vi "Obtain Request Events.vi"(8 "error in":errorcluster, 10 "Create New? (F)":bool) -> (0 "error out":errorcluster, 2 "Sequencer Request Events":T1)   [LabVIEW 2025, in "Sequencer.lvlib"]
doc: "This VI Obtains/Creates the Requests events that will be used for other modules to communicate with the module that owns this VI. These Requests events will be accessed only via Public API methods for this module.\n\n<b>NOTE</b>: The contents of this VI are automatically generated and modified by the <b>Tools > DQMH Consortium > DQMH</b> utilities. Consider using those utilities instead of making your own modifications to this VI.\n_____\nBased on DQMH Dev Tools: Project Template 7.1.2.1547."
uses:
  Sequencer.lvlib
  Request Events--cluster.ctl
  Stop Argument--cluster.ctl
  Show Panel Argument--cluster.ctl
  Hide Panel Argument--cluster.ctl
  Show Diagram Argument--cluster.ctl
  Get Module Execution Status Argument--cluster.ctl
  Get Modules Argument--cluster.ctl
  Get Modules (Reply Payload)--cluster.ctl
  Home Argument--cluster.ctl
  Home (Reply Payload)--cluster.ctl
  Home Stepper Argument--cluster.ctl
  Home Stepper (Reply Payload)--cluster.ctl
  Go To Angle Argument--cluster.ctl
  Controls/Angle Indicator.ctl
  Controls/Motor Speed Slider.ctl
  Go To Angle (Reply Payload)--cluster.ctl
  Part Removal Position Argument--cluster.ctl
  Part Removal Position (Reply Payload)--cluster.ctl
  Torque Test Argument--cluster.ctl
  Controls/Sequencer/sequence array.ctl
  Controls/Sequencer/step cluster.ctl
  Torque Test (Reply Payload)--cluster.ctl
  Controls/Sequencer/results array.ctl
  Controls/Sequencer/results cluster.ctl
panel:
  # "NOTE: The contents of this VI are automatically generated and modified by the Tools > DQMH Consortium > DQMH utilities. Consider using those utilities instead of making your own modifications to this VI."
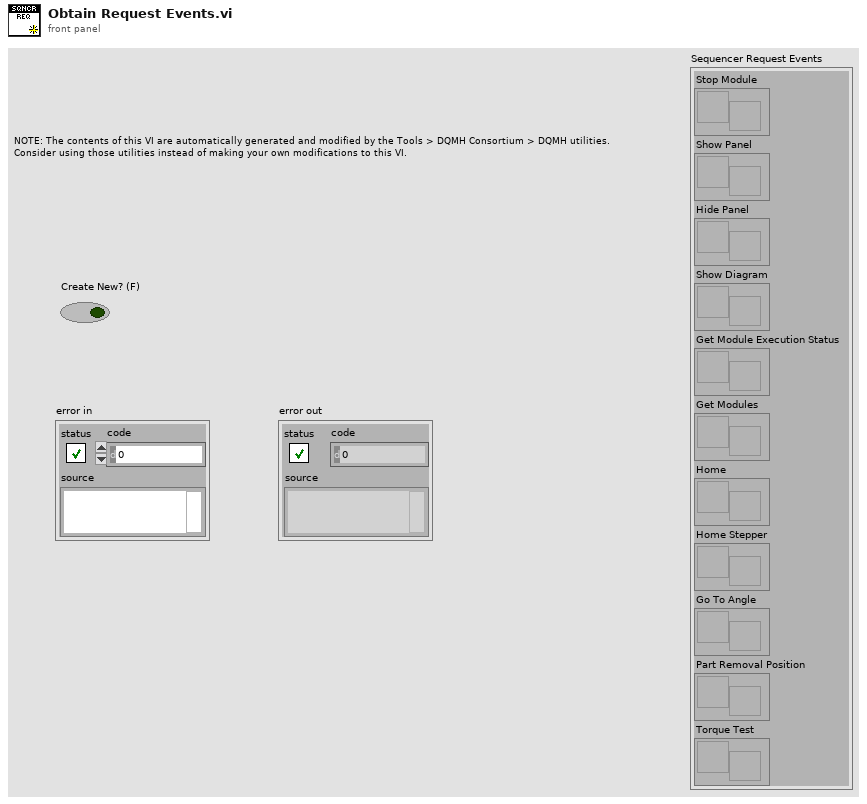
[diagram p1: front panel]
types:
  T1 = typedef "Sequencer.lvlib/Request Events--cluster.ctl" = cluster{"Stop Module":refnum<user-event>, "Show Panel":refnum<user-event>, "Hide Panel":refnum<user-event>, "Show Diagram":refnum<user-event>, "Get Module Execution Status":refnum<user-event>, "Get Modules":refnum<user-event>, "Home":refnum<user-event>, "Home Stepper":refnum<user-event>, "Go To Angle":refnum<user-event>, "Part Removal Position":refnum<user-event>, "Torque Test":refnum<user-event>}
  T2 = typedef "Sequencer.lvlib/Torque Test Argument--cluster.ctl" = cluster{"Module ID":i32, "Array 2":T3, "Speed [rpm]":T5, "On Time [ms]":dbl, "Wait Notifier":refnum<notifier>, "wait for reply":bool}
  T3 = typedef "sequence array.ctl" = T4[]
  T4 = typedef "step cluster.ctl" = cluster{"Angle Min [°]":dbl, "Angle Max [°]":dbl, "Torque Min [oz-in]":dbl, "Torque Max [oz-in]":dbl}
  T5 = typedef "Motor Speed Slider.ctl" = dbl
  T6 = typedef "Sequencer.lvlib/Part Removal Position Argument--cluster.ctl" = cluster{"Module ID":i32, "Wait Notifier":refnum<notifier>, "wait for reply":bool}
  T7 = typedef "Sequencer.lvlib/Go To Angle Argument--cluster.ctl" = cluster{"Module ID":i32, "Angle":T8, "Speed [rpm]":T5, "Wait Notifier":refnum<notifier>, "wait for reply":bool}
  T8 = typedef "Angle Indicator.ctl" = dbl
  T9 = typedef "Sequencer.lvlib/Home Stepper Argument--cluster.ctl" = cluster{"Module ID":i32, "Wait Notifier":refnum<notifier>, "wait for reply":bool}
  T10 = typedef "Sequencer.lvlib/Home Argument--cluster.ctl" = cluster{"Module ID":i32, "Wait Notifier":refnum<notifier>, "wait for reply":bool}
  T11 = typedef "Sequencer.lvlib/Get Modules Argument--cluster.ctl" = cluster{"Module ID":i32, "Modules":cluster{"Module IDs":i32[], "Module Names":string[]}, "Wait Notifier":refnum<notifier>, "wait for reply":bool}
  T12 = typedef "Sequencer.lvlib/Get Module Execution Status Argument--cluster.ctl" = cluster{"Module ID":i32, "Running?":bool}
  T13 = typedef "Sequencer.lvlib/Show Diagram Argument--cluster.ctl" = cluster{"Module ID":i32, "Debug?":bool}
  T14 = typedef "Sequencer.lvlib/Show Panel Argument--cluster.ctl" = cluster{"Module ID":i32, "Show Panel?":bool}
  T15 = typedef "Sequencer.lvlib/Hide Panel Argument--cluster.ctl" = cluster{"Module ID":i32, "Hide Panel?":bool}
  T16 = typedef "Sequencer.lvlib/Stop Argument--cluster.ctl" = cluster{"Module ID":i32, "Origin":string, "Exit via Stop Module Req?":bool, "Wait for Module to stop?":bool}
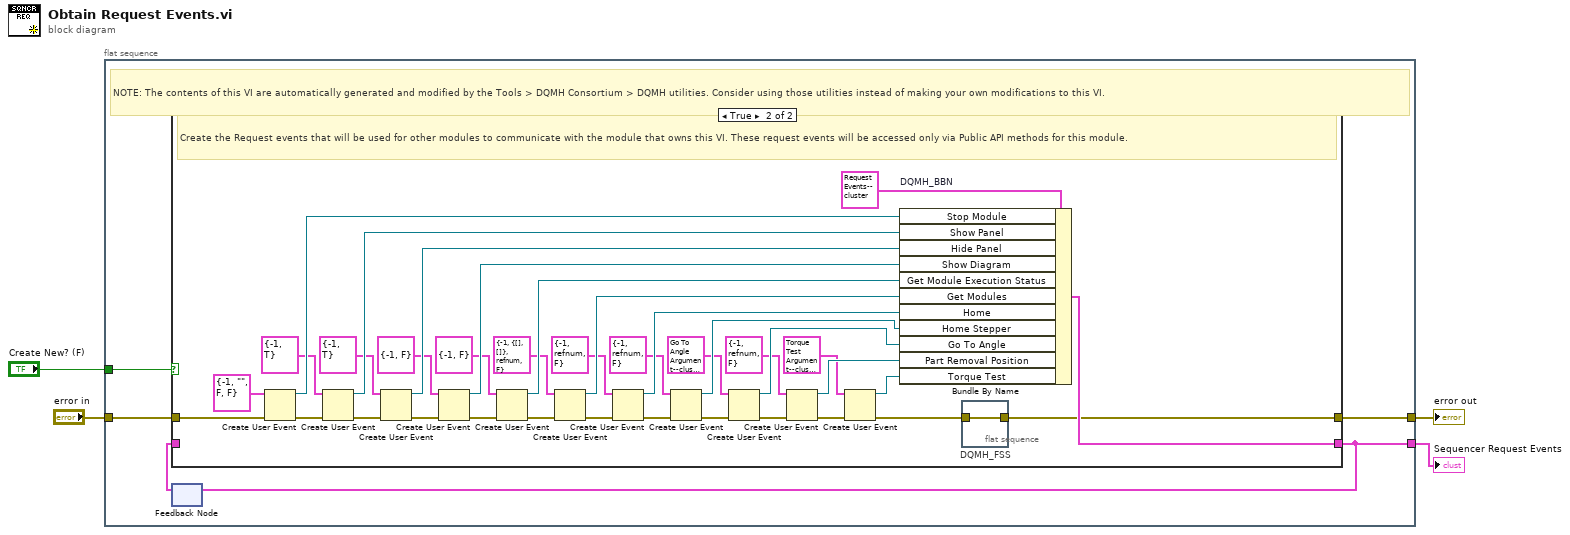
[diagram p0: block diagram]
diagram:
  n1 = flat-sequence {
    tunnel: [w9] -> w4
    tunnel: "error in" -> [w8]
    tunnel: [w6] -> w2
    tunnel: "Create New? (F)" -> [w5]
    frame #0 {
      # "NOTE: The contents of this VI are automatically generated and modified by the Tools > DQMH Consortium > DQMH utilities. Consider using those utilities instead of making your own modifications to this VI."
      n2 = feedback #1() -> (w7:T1)  [unwired: 1 in]
      n3 = case shown="True" w5 {
        tunnel: [w10 w36] -> w9
        tunnel: w8 -> [w10 w48]
        tunnel: [w11 w45] -> w6
        tunnel: w7 -> [w11 _]
        frame False {
        }
        frame True {
          # "Create the Request events that will be used for other modules to communicate with the module that owns this VI. These request events will be accessed only via Public API methods for this module."
          n4 = Create User Event(user event datatype=T16 {"Module ID"=-1, "Origin"="", "Exit via Stop Module Req?"=FALSE, "Wait for Module to stop?"=FALSE} ("Stop Argument"), error in=w48) -> (user event=w46:refnum<user-event>, error out=w43:errorcluster)
          n5 = Create User Event(user event datatype=T14 {"Module ID"=-1, "Show Panel?"=TRUE} ("Show Panel Argument"), error in=w43) -> (user event=w42:refnum<user-event>, error out=w40:errorcluster)
          n6 = Create User Event(user event datatype=T15 {"Module ID"=-1, "Hide Panel?"=TRUE} ("Hide Panel"), error in=w40) -> (user event=w39:refnum<user-event>, error out=w38:errorcluster)
          n7 = Create User Event(user event datatype=T13 {"Module ID"=-1, "Debug?"=FALSE} ("Show Diagram Argument"), error in=w38) -> (user event=w34:refnum<user-event>, error out=w35:errorcluster)
          n8 = Create User Event(user event datatype=T12 {"Module ID"=-1, "Running?"=FALSE} ("Get Module Execution Status Argument"), error in=w35) -> (user event=w31:refnum<user-event>, error out=w32:errorcluster)
          n9 = Create User Event(user event datatype=T11 {"Module ID"=-1, "Modules"={"Module IDs"=[], "Module Names"=[]}, "Wait Notifier"=refnum, "wait for reply"=FALSE} ("Get Modules Argument"), error in=w32) -> (user event=w28:refnum<user-event>, error out=w29:errorcluster)
          n10 = Create User Event(user event datatype=T10 {"Module ID"=-1, "Wait Notifier"=refnum, "wait for reply"=FALSE} ("Home Argument"), error in=w29) -> (user event=w25:refnum<user-event>, error out=w26:errorcluster)
          n11 = Create User Event(user event datatype=T9 {"Module ID"=-1, "Wait Notifier"=refnum, "wait for reply"=FALSE} ("Home Stepper Argument"), error in=w26) -> (user event=w22:refnum<user-event>, error out=w23:errorcluster)
          n12 = Create User Event(user event datatype=T7 {"Module ID"=-1, "Angle"=0.0, "Speed [rpm]"=9.818181818181818, "Wait Notifier"=refnum, "wait for reply"=FALSE} ("Go To Angle Argument"), error in=w23) -> (user event=w19:refnum<user-event>, error out=w20:errorcluster)
          n13 = Create User Event(user event datatype=T6 {"Module ID"=-1, "Wait Notifier"=refnum, "wait for reply"=FALSE} ("Part Removal Position Argument"), error in=w20) -> (user event=w16:refnum<user-event>, error out=w17:errorcluster)
          n14 = Create User Event(user event datatype=T2 {"Module ID"=-1, "Array 2"=[], "Speed [rpm]"=9.818181818181818, "On Time [ms]"=0.0, "Wait Notifier"=refnum, "wait for reply"=FALSE} ("Torque Test Argument"), error in=w17) -> (user event=w13:refnum<user-event>, error out=w14:errorcluster)
          n15 = Bundle By Name "DQMH_BBN"(cluster=T1 {"Stop Module"=refnum, "Show Panel"=refnum, "Hide Panel"=refnum, "Show Diagram"=refnum, "Get Module Execution Status"=refnum, "Get Modules"=refnum, "Home"=refnum, "Home Stepper"=refnum, "Go To Angle"=refnum, "Part Removal Position"=refnum, "Torque Test"=refnum} ("output cluster"), "Stop Module"=w46, "Show Panel"=w42, "Hide Panel"=w39, "Show Diagram"=w34, "Get Module Execution Status"=w31, "Get Modules"=w28, "Home"=w25, "Home Stepper"=w22, "Go To Angle"=w19, "Part Removal Position"=w16, "Torque Test"=w13) -> (w45:T1)
          n16 = flat-sequence "DQMH_FSS" {
            tunnel: w14 -> [w49]
            tunnel: [w49] -> w36
            frame #0 {
            }
          }
        }
      }
      n17 = feedback-in #1(w6) -> ()
    }
  }
  "Sequencer Request Events" <- w2
  "error out" <- w4
